vi "Cleanup.vi"(8 "error in (no error)":errorcluster, 11 "Node in":refnum<class "bt_Decorator.lvclass">) -> (0 "error out":errorcluster, 3 "Node out":refnum<class "bt_Decorator.lvclass">)   [LabVIEW 2021, in "BT.lvlib" / "bt_Decorator.lvclass"]
uses:
  bt_Decorator.lvclass
  bt_Decorator.lvclass/bt_Decorator.ctl
  abs_Node/bt_Node.lvclass
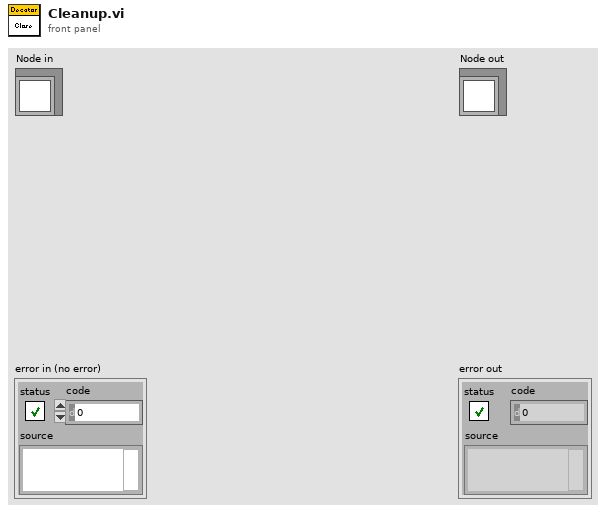
[diagram p1: front panel]
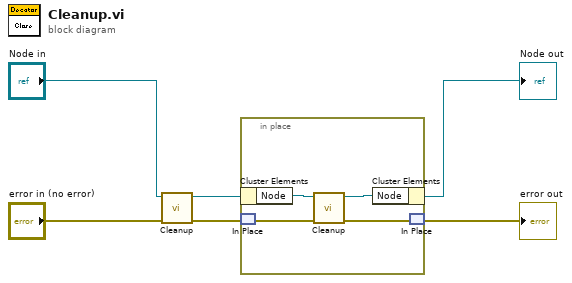
[diagram p0: block diagram]
diagram:
  n1 = call-parent "Cleanup.vi"("error in (no error)"="error in (no error)", "Node in"="Node in") -> ("error out"=w1:errorcluster, "Node out"=w2:refnum<class "bt_Decorator.lvclass">)  [unwired: 8 in]
  n2 = in-place {
    n3 = in-place-cluster #1(w2) -> ("Node"=w10:refnum<class "bt_Node.lvclass">)
    n4 = in-place-match #2(w1) -> (w8:errorcluster)
    n5 = call-dynamic "Cleanup.vi"("error in (no error)"=w8, "Node in"=w10) -> ("error out"=w7:errorcluster, "Node out"=w9:refnum<class "bt_Node.lvclass">)  [unwired: 8 in]
    n6 = in-place-cluster #1("Node"=w9) -> (→"Node out":refnum<class "bt_Decorator.lvclass">)
    n7 = in-place-match #2(w7) -> (→"error out":errorcluster)
  }
